vi "Complete Tool Entry.vi"(6 "terminals":T1(array[cluster]), 7 "outputs":T2(array[cluster]), 8 "error in":errorcluster, 9 "annotations":T3, 10 "title":string, 11 "tool entry":string) -> (0 "error out":errorcluster, 3 "tool entry out":string)   [LabVIEW 2020, in "MCP Server.lvlib"]
doc: "Completes the tools/list entry of one tool with what Add Tool.vi was given beyond the VI itself, and with the schema of its outputs.\n\n- title: the entry's title is replaced by title. When title is empty the entry has no title.\n- annotations: every hint that is set (true or false) goes into annotations under its MCP name (readOnlyHint, destructiveHint, idempotentHint, openWorldHint). Hints that are not set are left out, so the client applies the MCP default. When no hint is set the entry has no annotations.\n- outputSchema: an object schema with one property per output of the tool that is not a picture, named like the outputs in structuredContent and in the text of tools/call, and all of them in required. Each property is the type schema of the indicator (sub type from Get Connector Pane Info.vi, made by LV Type To JSON Schema.vi and Add Control Details To Schema.vi) merged over its MCP type and description, without default. A tool without such outputs gets no outputSchema.\n\nWith an error in the entry is passed through unchanged."
uses:
  MCP Server.lvlib
  <vilib>/JDP Science/JSONtext/JSONtext.lvlib
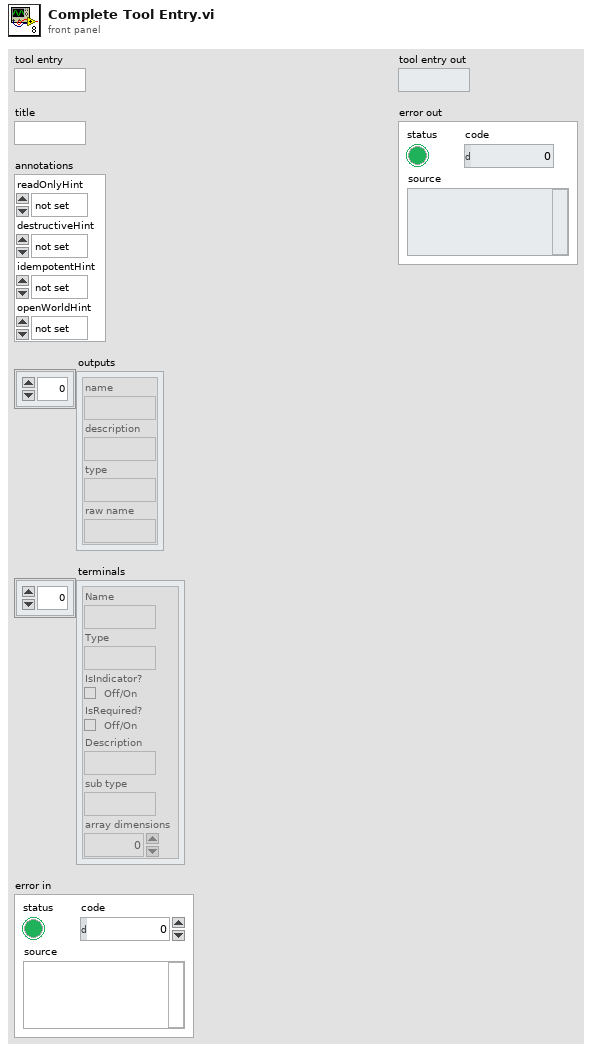
[diagram p1: front panel]
types:
  T1 = cluster{"Name":string, "Type":string, "IsIndicator?":bool, "IsRequired?":bool, "Description":string, "sub type":string, "array dimensions":i32}[]
  T2 = cluster{"name":string, "description":string, "type":string, "raw name":string}[]
  T3 = cluster{"readOnlyHint":enum16{"not set", "true", "false"}, "destructiveHint":enum16{"not set", "true", "false"}, "idempotentHint":enum16{"not set", "true", "false"}, "openWorldHint":enum16{"not set", "true", "false"}}
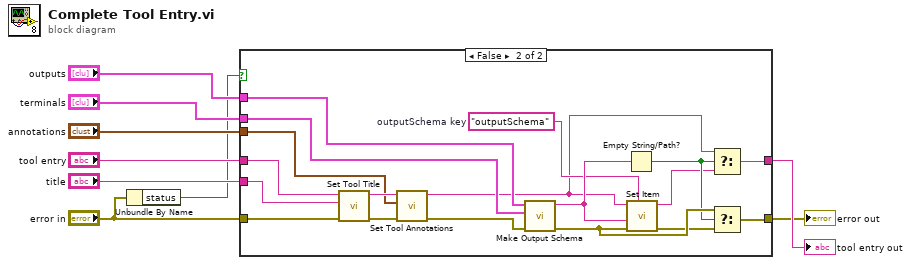
[diagram p0: block diagram]
diagram:
  n1 = Unbundle By Name("error in") -> ("status"=w3:bool)
  n2 = case shown="False" w3 {
    tunnel: "tool entry" -> [w11 w29]
    tunnel: "title" -> [_ w28]
    tunnel: "annotations" -> [_ w25]
    tunnel: "outputs" -> [_ w23]
    tunnel: "terminals" -> [_ w22]
    tunnel: "error in" -> [w10 w27]
    tunnel: [w11 w13] -> w2
    tunnel: [w10 w12] -> w1
    frame True {
    }
    frame False {
      w19 = "outputSchema"  # outputSchema key
      n3 = call "Set Tool Title.vi"("error in"=w27, "title"=w28, "tool entry"=w29) -> ("error out"=w24:errorcluster, "tool entry out"=w26:string)  [unwired: 7 in]
      n4 = call "Set Tool Annotations.vi"("error in"=w24, "annotations"=w25, "tool entry"=w26) -> ("error out"=w21:errorcluster, "tool entry out"=w16:string)  [unwired: 7 in]
      n5 = call "Make Output Schema.vi"("error in"=w21, "terminals"=w22, "outputs"=w23) -> ("error out"=w18:errorcluster, "output schema"=w20:string)  [unwired: 7 in]
      n6 = Empty String/Path?(string/path=w20) -> (empty?=w15:bool)
      n7 = call <vilib>:"Set Item.vi"("$Path or Item Name"=w19, "error in (no error)"=w18, "JSON to Insert"=w20, "JSON"=w16) -> ("error out"=w17:errorcluster, "<JSON>"=w14:string)  [unwired: 4 in, 1 out]
      n8 = Select(t=w16, s=w15, f=w14) -> (s? t:f=w13:string)
      n9 = Select(t=w18, s=w15, f=w17) -> (s? t:f=w12:errorcluster)
    }
  }
  "tool entry out" <- w2
  "error out" <- w1
